vi "Runtest - Data Structure (FGV).vi"(7 "Action":T10=enum."Write", 8 "error in (no error)":errorcluster, 11 "Cluster In":T1={"Test Plan"=[], "PlanRow"=0, "Device Name"=[], "Timeout"=-1, "Start?"=FALSE, "Pause?"=FALSE, "IP Address"=[], "LogRow"=0, "Logtype"=0, "Log Elapse"=0.0, "Data"={"Station"="", "Sample ID"="", "Job No"="", "Job Description"="", "Filename"="", "Test Type"=0, "Speciment No"="", "Depth"="", "Height"="", "Diameter/Length"="", "Weight"="", "Test Parameter"="", "Station[]"=[], "Edit Pos"={"Row"=0, "Column"=0}, "Edit Pos Prev"={"Row"=0, "Column"=0}, "Area"="", "Path"="", "sample_id"=""}, "Stop log?"=FALSE, "tdms"=refnum, "Sensor Data"=[], "Start time"=timestamp(0 s since 1904-01-01), "Prev Log Elapse"=0, "Plot"=0, "X-Axis"=[0, 0, 0, 0], "Y-Axis"=[0, 0, 0, 0], "XY"=[], "End Stage?"=FALSE, "1run"=FALSE, "Condition"=[], "Start Con"=TRUE, "Log Con"=FALSE, "Stop Con"=FALSE, "Start Elapse"=0.0, "Start Load"=0.0, "Motor"=0, "StartRow"=0, "number log"=0, "Dir"=FALSE, "Start time test"=timestamp(0 s since 1904-01-01), "Auto"=FALSE, "Check return?"=FALSE, "Inv"={"M"=[], "Bool"=[]}, "tdms temp"=refnum, "Zero?"=FALSE, "Plot Timer"=0.0, "1st Run"=FALSE, "TDMS Path"=path "", "MaxLoad"=0.0, "Log Timer"=[], "Test Type"=0, "Log Sensor"=[], "Save?"=FALSE, "1st Log"=FALSE, "Y-Axis 2"=[], "On Y-Axis 2"=FALSE, "Decimal"=[], "Init"={"PWP TS"=0.0, "Load TS"=0.0, "Volume TS"=0.0, "Disp TS"=0.0, "CP"=0.0, "Vol In"=0.0, "Vol Out"=0.0, "Load UCT"=0.0, "Disp UCT"=0.0, "PWP Sat"=0.0, "CP Sat"=0.0, "Volume IsoCons"=0.0, "PWP IsoCons"=0.0, "PWP TUU"=0.0, "Load TUU"=0.0, "Volume TUU"=0.0, "Disp TUU"=0.0, "Load Cons"=0.0, "Disp Cons"=0.0, "Volume Sat"=0.0, "Vertical Load SB"=0.0, "Vertical Disp SB"=0.0, "H Disp SB"=0.0, "H Load SB"=0.0, "PWP BC"=0.0, "CP BC"=0.0, "PWP Sat Step"=0.0, "CP Sat Step"=0.0, "Volume Sat Step"=0.0, "PWP Sat Ramp"=0.0, "CP Sat Ramp"=0.0, "Volume Sat Ramp"=0.0}, "Calc"={"TS"={"Change PWP"=0.0, "Change Vol"=0.0, "Axial Load"=0.0, "CiL"=0.0, "Deviator"=0.0, "Axial Strain"=0.0, "MaxDeviator"=0.0, "SS"=0.0, "CAS"=0.0}, "TUU"={"Change PWP"=0.0, "Axial Load"=0.0, "CiL"=0.0, "Deviator"=0.0, "Axial Strain"=0.0, "MaxDeviator"=0.0}, "Sat"={"B Value"=0.0, "PWP Diss"=0.0, "CPP"=0.0, "CV"=0.0}, "Per"={"Change Vol In"=0.0, "Change Vol Out"=0.0, "Mean Vol"=0.0, "Gradient Pressure"=0.0, "Outlet Flow"=0.0, "Inlet Flow"=0.0, "I X1"=0.0, "I X2"=0.0, "I Y1"=0.0, "I Y2"=0.0, "O X1"=0.0, "O X2"=0.0, "O Y1"=0.0, "O Y2"=0.0}, "Step Cons"={"V Stress"=0.0, "H Settlement"=0.0, "Total H Settle"=0.0, "Prev Total H"=0.0}, "UCT"={"ALC"=0.0, "H Change"=0.0, "Deviator"=0.0, "Axial Strain"=0.0, "V Stress"=0.0, "MaxDeviator"=0.0}, "ISO Cons"={"CPP"=0.0, "PWP Diss"=0.0, "CV"=0.0, "VS"=0.0}, "SB"={"Speci LenC"=0.0, "Shear Strain"=0.0, "H LC"=0.0, "Normal Stress"=0.0, "Shear Stress"=0.0, "MaxShear"=0.0}, "BC"={"B Value"=0.0, "PWP Diss"=0.0, "CPP"=0.0, "CV"=0.0}, "Sat Step"={"B Value"=0.0, "PWP Diss"=0.0, "CPP"=0.0, "CV"=0.0}, "Sat Ramp"={"B Value"=0.0, "PWP Diss"=0.0, "CPP"=0.0, "CV"=0.0}}, "Device Index"=[], "Channel Index"=[], "http ref"=refnum, "fileid"="", "Step Cons"={"V Stress"=0.0, "H Settlement"=0.0}, "RunTest"=FALSE, "Graph Last"=0, "Init?"=FALSE, "Datalog"=[], "Start"={"Cons"={"VS"=0.0, "Delay"=FALSE, "No Delay"=0.0}, "Sat"={"CP"=0.0, "BP"=0.0, "StartBP"=FALSE, "Target CP"=FALSE, "Target BP"=FALSE}, "Iso"={"Select"=0.0, "BP"=0.0, "IC2"=0.0, "IC3"=0.0, "IC4"=0.0, ". IC6"=FALSE, "IC6"=0.0, "IC6-2"=0.0, "Time Cond"=0.0, "Last PWP"=0.0, "Target CP"=FALSE, "Target BP"=FALSE, "NewCP"=0.0, "NewBP"=0.0, "Noti CP"=FALSE, "Noti BP"=FALSE, "Noti PWP"=FALSE, "PrevSatBP"=0.0}, "TS"={"SS"=0.0, "Engage"=FALSE, "ES"=0.0, "LC"=0.0, "PreStart"=FALSE, "Trig SS"=FALSE, "Drain"=0.0, "Select"=0, "Max SS ."=FALSE, "MaxSS"=0.0}, "TUU"={"SS"=0.0, "Engage"=FALSE, "ES"=0.0, "LC"=0.0, "PreStart"=FALSE, "Trig SS"=FALSE, "CP"=0.0, "Delay Value"=0.0, "Delay"=FALSE, "CP PID"=FALSE}, "UCT"={"SS"=0.0, "Engage"=FALSE, "ES"=0.0, "LC"=0.0, "PreStart"=FALSE, "Trig SS"=FALSE}, "Enable?"=FALSE, "SB"={"SS"=0.0, "Engage"=FALSE, "ES"=0.0, "LC"=0.0, "PreStart"=FALSE, "Trig SS"=FALSE, "VS"=0.0, "Delay Value"=0.0, "Delay"=FALSE, "VS PID"=FALSE}, "Perm"={"DP"=0.0}, "BC"={"CP"=0.0, "Target CP"=FALSE, "Target BP"=FALSE, "CP Inc"=0.0, "CP .Init"=FALSE, "CP Init"=0.0, "1st BC"=FALSE}, "Sat (Step)"={"Select"=0.0, "CP"=0.0, "BP"=0.0, "EP"=0.0, "StartCP"=FALSE, "Target CP"=FALSE, "Target BP"=FALSE}, "Sat (Ramp)"={"Select"=0.0, "CP"=0.0, "BP"=0.0, "EP"=0.0, "StartCP"=FALSE, "Target CP"=FALSE, "Target BP"=FALSE, "Time Rate"=0}}, "Stop"={"Cons"={"Select"=0, "Disp"=0.0, "Time"=0.0, "Time2"=0.0, "Disp 2"=0.0, "Time Cond"=0.0, "Last Disp"=0.0, "Swell"=FALSE, "T50,90,100"={"t50_x_min"=0.0, "t50_y_value"=0.0, "t90_x_min"=0.0, "t90_y_value"=0.0, "t100_x_min"=0.0, "t100_y_value"=0.0, "target_column"="", "test_type"="", "error"=""}}, "Sat"={"Select"=0, "PP"=0.0, "Time"=0.0, "VC"=0.0, "Time2"=0.0, "Time Cond"=0.0, "Last PP"=0.0, ".B"=FALSE, "B"=0.0, "Last Vc"=0.0, "Time Cond 2"=0.0, "Time3"=0.0, "Time Cond 3"=0.0, "B Achieve"=FALSE, "PP Achieve"=FALSE, "VC Achieve"=FALSE, "Max Achieve"=FALSE, "CP Check"=0.0, "Skip Next"=FALSE, "B Achieve Stage"=0, ".CP Check"=FALSE}, "Iso"={"PP"=0.0, "Time"=0.0, "VC"=0.0, "Time2"=0.0, "Time Cond"=0.0, "Last Vc"=0.0, ".PP"=FALSE, "Time Cond 2"=0.0, "Select"=0, "BS"={"t50_x_min"=0.0, "t50_y_value"=0.0, "t90_x_min"=0.0, "t90_y_value"=0.0, "t100_x_min"=0.0, "t100_y_value"=0.0, "target_column"="", "test_type"="", "error"=""}, "Final VC"=0.0, "ASTM"={"t50_x_min"=0.0, "t50_y_value"=0.0, "t90_x_min"=0.0, "t90_y_value"=0.0, "t100_x_min"=0.0, "t100_y_value"=0.0, "target_column"="", "test_type"="", "error"=""}, "ASTM Log"={"t50_x_min"=0.0, "t50_y_value"=0.0, "t90_x_min"=0.0, "t90_y_value"=0.0, "t100_x_min"=0.0, "t100_y_value"=0.0, "target_column"="", "test_type"="", "error"=""}, "PP Achieve"=FALSE, "VC Achieve"=FALSE}, "TS"={"Axial"=0.0, ".MaxDev"=FALSE, "MaxDev Value"=0.0, "Return"=FALSE, "Reset"=FALSE, "Prev Time"=0.0, "PostStop Run"=FALSE, "CP Stop"=FALSE, "BP Stop"=FALSE, "PostStop Trig"=FALSE, "Reset Value"=0.0, "BPTrig"=FALSE, "CPTrig"=FALSE, "VLCTrig"=FALSE, "CAxial"=0.0, "Select"=0}, "TUU"={"Axial"=0.0, ".MaxDev"=FALSE, "MaxDev Value"=0.0, "Return"=FALSE, "Reset"=FALSE, "Prev Time"=0.0, "PostStop Run"=FALSE, "CP Stop"=FALSE, "BP Stop"=FALSE, "PostStop Trig"=FALSE, "Reset Value"=0.0, "BPTrig"=FALSE, "CPTrig"=FALSE, "VLCTrig"=FALSE}, "UCT"={"Axial"=0.0, ".MaxDev"=FALSE, "MaxDev Value"=0.0, "Return"=FALSE, "Reset"=FALSE, "Prev Time"=0.0, "PostStop Run"=FALSE, "CP Stop"=FALSE, "BP Stop"=FALSE, "PostStop Trig"=FALSE}, "Enable?"=FALSE, "SB"={"Shear"=0.0, ".MaxShear"=FALSE, "MaxShear Value"=0.0, "Return"=FALSE, "Reset"=FALSE, "Prev Time"=0.0, "PostStop Run"=FALSE, "CP Stop"=FALSE, "BP Stop"=FALSE, "PostStop Trig"=FALSE, "Reset Value"=0.0, "BPTrig"=FALSE, "CPTrig"=FALSE, "VLCTrig"=FALSE}, "Perm"={"Max Time"=FALSE, "Reset"=FALSE, "PostStop Run"=FALSE, "Ratio"=FALSE, "Reset Value"=0.0, "Time"=0.0, "RatioTime"=0.0, "RatioMore"=0.0, "RatioLess"=0.0, "Time Cond"=0.0, "Time Cond 2"=0.0, "Prev IF"=0.0, "Prev OF"=0.0, "PostStop Trig"=FALSE, "BP Trig"=FALSE, "DP Stop"=FALSE, "BP Stop"=FALSE, "CP Stop"=FALSE, "CP Trig"=FALSE}, "SP"={".Max Time"=FALSE, ".Time"=FALSE, "Time"=0.0, "MaxTime"=0.0, "Time Cond"=0.0, "Max Time Cond"=0.0, "Stress"=0.0}, "BC"={"Select"=0, "PP"=0.0, "Time"=0.0, "Time Cond"=0.0, "Last PP"=0.0, ".B"=FALSE, "B"=0.0, "Time 2"=0.0, "Time Cond 2"=0.0, "B Achieve"=FALSE, "PP Achieve"=FALSE, "Max Achieve"=FALSE, "CP Check"=0.0, "Skip Next"=FALSE, "B Achieve Stage"=0, ".CP Check"=FALSE}, "Sat (Step)"={"Select"=0, "PP"=0.0, "Time"=0.0, "VC"=0.0, "Time2"=0.0, "Time Cond"=0.0, "Last PP"=0.0, ".B"=FALSE, "B"=0.0, "Last Vc"=0.0, "Time Cond 2"=0.0, "Time3"=0.0, "Time Cond 3"=0.0, "B Achieve"=FALSE, "PP Achieve"=FALSE, "VC Achieve"=FALSE, "Max Achieve"=FALSE, "CP Check"=0.0, "Skip Next"=FALSE, "B Achieve Stage"=0}, "Sat (Ramp)"={"Select"=0, "PP"=0.0, "Time"=0.0, "VC"=0.0, "Time2"=0.0, "Time Cond"=0.0, "Last PP"=0.0, ".B"=FALSE, "B"=0.0, "Last Vc"=0.0, "Time Cond 2"=0.0, "Time3"=0.0, "Time Cond 3"=0.0, "B Achieve"=FALSE, "PP Achieve"=FALSE, "VC Achieve"=FALSE, "Max Achieve"=FALSE, "CP Check"=0.0, "Skip Next"=FALSE, "B Achieve Stage"=0}}, "Running?"=FALSE, "StartTime"=0.0, "Log Prev Time"=0.0, "KeyName"=[], "Test RunTime"=0.0, "Log Prev Axial"=0.0, "M Event"=[], "Last Log"=FALSE, "popup"=FALSE, "PreStart UU"=FALSE, "PreStart Sat"=FALSE, "PreStart BC"=FALSE, "PreStart Sat Step"=FALSE, "PreStart Sat Ramp"=FALSE, "Prev Sat IP"=""} {"M Event" items=["Stop", "Running", "PID", "Up Limit", "Down Limit", "Load Limit"]; "Test Type" items=["Please Select", "Triaxial Shear", "Triaxial UU", "Shearbox", "Permeability", "Consolidation (Stepped Loading)/Swelling", "Saturation (Incremental)", "User Defined", "UCT", "Isotropic Consolidation", "Swelling Pressure", "B-Check", "Saturation (Step Increment)", "Saturation (Ramp)"]; "Data"."Test Type" items=["Please Select", "Triaxial Shear", "Triaxial UU", "Shearbox", "Permeability", "Consolidation (Stepped Loading)/Swelling", "Saturation (Incremental)", "User Defined", "UCT", "Isotropic Consolidation", "Swelling Pressure", "B-Check", "Saturation (Step Increment)", "Saturation (Ramp)"]}) -> (0 "error out":errorcluster, 3 "Cluster Out":T1 {"M Event" items=["Stop", "Running", "PID", "Up Limit", "Down Limit", "Load Limit"]; "Test Type" items=["Please Select", "Triaxial Shear", "Triaxial UU", "Shearbox", "Permeability", "Consolidation (Stepped Loading)/Swelling", "Saturation (Incremental)", "User Defined", "UCT", "Isotropic Consolidation", "Swelling Pressure", "B-Check", "Saturation (Step Increment)", "Saturation (Ramp)"]; "Data"."Test Type" items=["Please Select", "Triaxial Shear", "Triaxial UU", "Shearbox", "Permeability", "Consolidation (Stepped Loading)/Swelling", "Saturation (Incremental)", "User Defined", "UCT", "Isotropic Consolidation", "Swelling Pressure", "B-Check", "Saturation (Step Increment)", "Saturation (Ramp)"]})   [LabVIEW 2019]
uses:
  Controls/FGV States.ctl
  Controls/RunTest - Data Structure.ctl
  Controls/Test Panel - Data Structure.ctl
  Controls/Station - Test Type.ctl
  <vilib>/Utility/miscctls.llb/LVRowAndColumnTypeDef.ctl
  Controls/RunTest - Calculate Data.ctl
  <vilib>/httpClient/ClientHandle.ctl
  Controls/RunTest - Start Condition.ctl
  Controls/RunTest - Stop Condition.ctl
  Controls/UDP - Event.ctl
  <vilib>/httpClient/LabVIEWHTTPClient.lvlib
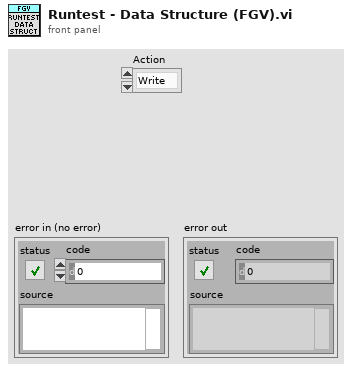
[diagram p1: front panel]
types:
  T1 = typedef "RunTest - Data Structure.ctl" = cluster{"Test Plan":string[], "PlanRow":i32, "Device Name":string[], "Timeout":i32, "Start?":bool, "Pause?":bool, "IP Address":string[], "LogRow":i32, "Logtype":u16, "Log Elapse":sgl, "Data":T2, "Stop log?":bool, "tdms":refnum<k34>, "Sensor Data":sgl[], "Start time":timestamp, "Prev Log Elapse":u32, "Plot":u16, "X-Axis":u16[], "Y-Axis":u16[], "XY":cluster{"X":dbl, "Y":dbl}[][], "End Stage?":bool, "1run":bool, "Condition":u16[], "Start Con":bool, "Log Con":bool, "Stop Con":bool, "Start Elapse":dbl, "Start Load":dbl, "Motor":i32, "StartRow":i32, "number log":i32, "Dir":bool, "Start time test":timestamp, "Auto":bool, "Check return?":bool, "Inv":cluster{"M":i32[], "Bool":bool[]}, "tdms temp":refnum<k34>, "Zero?":bool, "Plot Timer":dbl, "1st Run":bool, "TDMS Path":path, "MaxLoad":dbl, "Log Timer":sgl[], "Test Type":T3, "Log Sensor":string[], "Save?":bool, "1st Log":bool, "Y-Axis 2":u16[], "On Y-Axis 2":bool, "Decimal":u8[], "Init":cluster{"PWP TS":sgl, "Load TS":sgl, "Volume TS":sgl, "Disp TS":sgl, "CP":sgl, "Vol In":sgl, "Vol Out":sgl, "Load UCT":sgl, "Disp UCT":sgl, "PWP Sat":sgl, "CP Sat":sgl, "Volume IsoCons":sgl, "PWP IsoCons":sgl, "PWP TUU":sgl, "Load TUU":sgl, "Volume TUU":sgl, "Disp TUU":sgl, "Load Cons":sgl, "Disp Cons":sgl, "Volume Sat":sgl, "Vertical Load SB":sgl, "Vertical Disp SB":sgl, "H Disp SB":sgl, "H Load SB":sgl, "PWP BC":sgl, "CP BC":sgl, "PWP Sat Step":sgl, "CP Sat Step":sgl, "Volume Sat Step":sgl, "PWP Sat Ramp":sgl, "CP Sat Ramp":sgl, "Volume Sat Ramp":sgl}, "Calc":T5, "Device Index":i32[], "Channel Index":i32[], "http ref":T6, "fileid":string, "Step Cons":cluster{"V Stress":sgl, "H Settlement":sgl}, "RunTest":bool, "Graph Last":i32, "Init?":bool, "Datalog":bool[], "Start":T7, "Stop":T8, "Running?":bool, "StartTime":dbl, "Log Prev Time":dbl, "KeyName":string[], "Test RunTime":dbl, "Log Prev Axial":dbl, "M Event":T9[], "Last Log":bool, "popup":bool, "PreStart UU":bool, "PreStart Sat":bool, "PreStart BC":bool, "PreStart Sat Step":bool, "PreStart Sat Ramp":bool, "Prev Sat IP":string}
  T2 = typedef "Test Panel - Data Structure.ctl" = cluster{"Station":string, "Sample ID":string, "Job No":string, "Job Description":string, "Filename":string, "Test Type":T3, "Speciment No":string, "Depth":string, "Height":string, "Diameter/Length":string, "Weight":string, "Test Parameter":string, "Station[]":string[], "Edit Pos":T4, "Edit Pos Prev":T4, "Area":string, "Path":string, "sample_id":string}
  T3 = typedef "Station - Test Type.ctl" = u16
  T4 = typedef "LVRowAndColumnTypeDef.ctl" = cluster{"Row":i32, "Column":i32}
  T5 = typedef "RunTest - Calculate Data.ctl" = cluster{"TS":cluster{"Change PWP":sgl, "Change Vol":sgl, "Axial Load":sgl, "CiL":sgl, "Deviator":sgl, "Axial Strain":sgl, "MaxDeviator":sgl, "SS":sgl, "CAS":sgl}, "TUU":cluster{"Change PWP":sgl, "Axial Load":sgl, "CiL":sgl, "Deviator":sgl, "Axial Strain":sgl, "MaxDeviator":sgl}, "Sat":cluster{"B Value":sgl, "PWP Diss":sgl, "CPP":sgl, "CV":sgl}, "Per":cluster{"Change Vol In":sgl, "Change Vol Out":sgl, "Mean Vol":sgl, "Gradient Pressure":sgl, "Outlet Flow":sgl, "Inlet Flow":sgl, "I X1":sgl, "I X2":sgl, "I Y1":sgl, "I Y2":sgl, "O X1":sgl, "O X2":sgl, "O Y1":sgl, "O Y2":sgl}, "Step Cons":cluster{"V Stress":sgl, "H Settlement":sgl, "Total H Settle":sgl, "Prev Total H":sgl}, "UCT":cluster{"ALC":sgl, "H Change":sgl, "Deviator":sgl, "Axial Strain":sgl, "V Stress":sgl, "MaxDeviator":sgl}, "ISO Cons":cluster{"CPP":sgl, "PWP Diss":sgl, "CV":sgl, "VS":sgl}, "SB":cluster{"Speci LenC":sgl, "Shear Strain":sgl, "H LC":sgl, "Normal Stress":sgl, "Shear Stress":sgl, "MaxShear":sgl}, "BC":cluster{"B Value":sgl, "PWP Diss":sgl, "CPP":sgl, "CV":sgl}, "Sat Step":cluster{"B Value":sgl, "PWP Diss":sgl, "CPP":sgl, "CV":sgl}, "Sat Ramp":cluster{"B Value":sgl, "PWP Diss":sgl, "CPP":sgl, "CV":sgl}}
  T6 = typedef "LabVIEWHTTPClient.lvlib/ClientHandle.ctl" = refnum<k1>
  T7 = typedef "RunTest - Start Condition.ctl" = cluster{"Cons":cluster{"VS":dbl, "Delay":bool, "No Delay":dbl}, "Sat":cluster{"CP":dbl, "BP":dbl, "StartBP":bool, "Target CP":bool, "Target BP":bool}, "Iso":cluster{"Select":dbl, "BP":dbl, "IC2":dbl, "IC3":dbl, "IC4":dbl, ". IC6":bool, "IC6":dbl, "IC6-2":dbl, "Time Cond":dbl, "Last PWP":dbl, "Target CP":bool, "Target BP":bool, "NewCP":dbl, "NewBP":dbl, "Noti CP":bool, "Noti BP":bool, "Noti PWP":bool, "PrevSatBP":dbl}, "TS":cluster{"SS":dbl, "Engage":bool, "ES":dbl, "LC":dbl, "PreStart":bool, "Trig SS":bool, "Drain":dbl, "Select":u16, "Max SS .":bool, "MaxSS":dbl}, "TUU":cluster{"SS":dbl, "Engage":bool, "ES":dbl, "LC":dbl, "PreStart":bool, "Trig SS":bool, "CP":dbl, "Delay Value":dbl, "Delay":bool, "CP PID":bool}, "UCT":cluster{"SS":dbl, "Engage":bool, "ES":dbl, "LC":dbl, "PreStart":bool, "Trig SS":bool}, "Enable?":bool, "SB":cluster{"SS":dbl, "Engage":bool, "ES":dbl, "LC":dbl, "PreStart":bool, "Trig SS":bool, "VS":dbl, "Delay Value":dbl, "Delay":bool, "VS PID":bool}, "Perm":cluster{"DP":dbl}, "BC":cluster{"CP":dbl, "Target CP":bool, "Target BP":bool, "CP Inc":dbl, "CP .Init":bool, "CP Init":dbl, "1st BC":bool}, "Sat (Step)":cluster{"Select":dbl, "CP":dbl, "BP":dbl, "EP":dbl, "StartCP":bool, "Target CP":bool, "Target BP":bool}, "Sat (Ramp)":cluster{"Select":dbl, "CP":dbl, "BP":dbl, "EP":dbl, "StartCP":bool, "Target CP":bool, "Target BP":bool, "Time Rate":u32}}
  T8 = typedef "RunTest - Stop Condition.ctl" = cluster{"Cons":cluster{"Select":i32, "Disp":dbl, "Time":dbl, "Time2":dbl, "Disp 2":dbl, "Time Cond":dbl, "Last Disp":dbl, "Swell":bool, "T50,90,100":cluster{"t50_x_min":dbl, "t50_y_value":dbl, "t90_x_min":dbl, "t90_y_value":dbl, "t100_x_min":dbl, "t100_y_value":dbl, "target_column":string, "test_type":string, "error":string}}, "Sat":cluster{"Select":i32, "PP":dbl, "Time":dbl, "VC":dbl, "Time2":dbl, "Time Cond":dbl, "Last PP":dbl, ".B":bool, "B":dbl, "Last Vc":dbl, "Time Cond 2":dbl, "Time3":dbl, "Time Cond 3":dbl, "B Achieve":bool, "PP Achieve":bool, "VC Achieve":bool, "Max Achieve":bool, "CP Check":dbl, "Skip Next":bool, "B Achieve Stage":u32, ".CP Check":bool}, "Iso":cluster{"PP":dbl, "Time":dbl, "VC":dbl, "Time2":dbl, "Time Cond":dbl, "Last Vc":dbl, ".PP":bool, "Time Cond 2":dbl, "Select":i32, "BS":cluster{"t50_x_min":dbl, "t50_y_value":dbl, "t90_x_min":dbl, "t90_y_value":dbl, "t100_x_min":dbl, "t100_y_value":dbl, "target_column":string, "test_type":string, "error":string}, "Final VC":dbl, "ASTM":cluster{"t50_x_min":dbl, "t50_y_value":dbl, "t90_x_min":dbl, "t90_y_value":dbl, "t100_x_min":dbl, "t100_y_value":dbl, "target_column":string, "test_type":string, "error":string}, "ASTM Log":cluster{"t50_x_min":dbl, "t50_y_value":dbl, "t90_x_min":dbl, "t90_y_value":dbl, "t100_x_min":dbl, "t100_y_value":dbl, "target_column":string, "test_type":string, "error":string}, "PP Achieve":bool, "VC Achieve":bool}, "TS":cluster{"Axial":dbl, ".MaxDev":bool, "MaxDev Value":dbl, "Return":bool, "Reset":bool, "Prev Time":dbl, "PostStop Run":bool, "CP Stop":bool, "BP Stop":bool, "PostStop Trig":bool, "Reset Value":dbl, "BPTrig":bool, "CPTrig":bool, "VLCTrig":bool, "CAxial":dbl, "Select":i32}, "TUU":cluster{"Axial":dbl, ".MaxDev":bool, "MaxDev Value":dbl, "Return":bool, "Reset":bool, "Prev Time":dbl, "PostStop Run":bool, "CP Stop":bool, "BP Stop":bool, "PostStop Trig":bool, "Reset Value":dbl, "BPTrig":bool, "CPTrig":bool, "VLCTrig":bool}, "UCT":cluster{"Axial":dbl, ".MaxDev":bool, "MaxDev Value":dbl, "Return":bool, "Reset":bool, "Prev Time":dbl, "PostStop Run":bool, "CP Stop":bool, "BP Stop":bool, "PostStop Trig":bool}, "Enable?":bool, "SB":cluster{"Shear":dbl, ".MaxShear":bool, "MaxShear Value":dbl, "Return":bool, "Reset":bool, "Prev Time":dbl, "PostStop Run":bool, "CP Stop":bool, "BP Stop":bool, "PostStop Trig":bool, "Reset Value":dbl, "BPTrig":bool, "CPTrig":bool, "VLCTrig":bool}, "Perm":cluster{"Max Time":bool, "Reset":bool, "PostStop Run":bool, "Ratio":bool, "Reset Value":dbl, "Time":dbl, "RatioTime":dbl, "RatioMore":dbl, "RatioLess":dbl, "Time Cond":dbl, "Time Cond 2":dbl, "Prev IF":dbl, "Prev OF":dbl, "PostStop Trig":bool, "BP Trig":bool, "DP Stop":bool, "BP Stop":bool, "CP Stop":bool, "CP Trig":bool}, "SP":cluster{".Max Time":bool, ".Time":bool, "Time":dbl, "MaxTime":dbl, "Time Cond":dbl, "Max Time Cond":dbl, "Stress":dbl}, "BC":cluster{"Select":i32, "PP":dbl, "Time":dbl, "Time Cond":dbl, "Last PP":dbl, ".B":bool, "B":dbl, "Time 2":dbl, "Time Cond 2":dbl, "B Achieve":bool, "PP Achieve":bool, "Max Achieve":bool, "CP Check":dbl, "Skip Next":bool, "B Achieve Stage":u32, ".CP Check":bool}, "Sat (Step)":cluster{"Select":i32, "PP":dbl, "Time":dbl, "VC":dbl, "Time2":dbl, "Time Cond":dbl, "Last PP":dbl, ".B":bool, "B":dbl, "Last Vc":dbl, "Time Cond 2":dbl, "Time3":dbl, "Time Cond 3":dbl, "B Achieve":bool, "PP Achieve":bool, "VC Achieve":bool, "Max Achieve":bool, "CP Check":dbl, "Skip Next":bool, "B Achieve Stage":u32}, "Sat (Ramp)":cluster{"Select":i32, "PP":dbl, "Time":dbl, "VC":dbl, "Time2":dbl, "Time Cond":dbl, "Last PP":dbl, ".B":bool, "B":dbl, "Last Vc":dbl, "Time Cond 2":dbl, "Time3":dbl, "Time Cond 3":dbl, "B Achieve":bool, "PP Achieve":bool, "VC Achieve":bool, "Max Achieve":bool, "CP Check":dbl, "Skip Next":bool, "B Achieve Stage":u32}}
  T9 = typedef "UDP - Event.ctl" = u16
  T10 = typedef "FGV States.ctl" = enum16{"Read", "Write"}
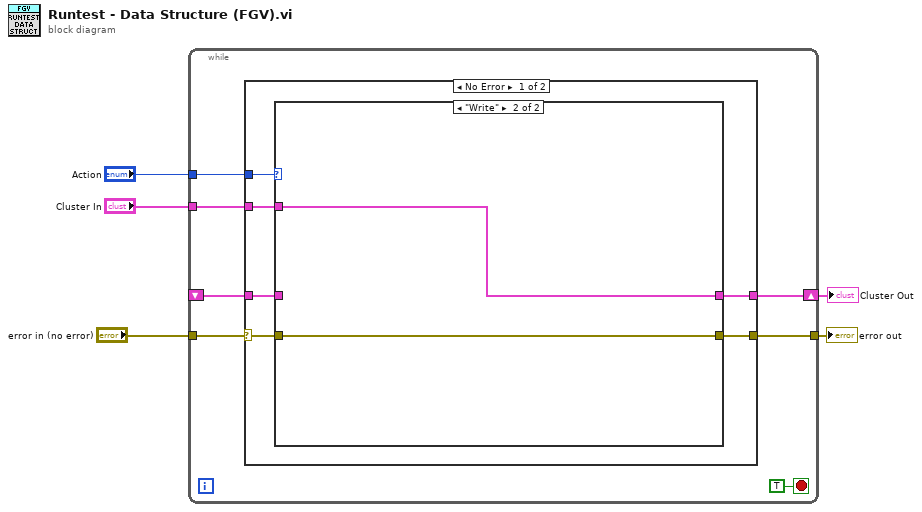
[diagram p0: block diagram]
diagram:
  n1 = while {
    tunnel: "Action" -> [w12]
    tunnel: "Cluster In" -> [w10]
    shift-right: [w11] -> w1
    shift-left: _ -> [w9]
    tunnel: "error in (no error)" -> [w7]
    tunnel: [w6] -> w3
    stop <- TRUE stop-if-true
    n2 = case shown="No Error" w7 {
      selector: w7 -> [w13 w23]
      tunnel: w12 -> [w18 _]
      tunnel: [w17 w24] -> w11
      tunnel: w10 -> [w16 _]
      tunnel: w9 -> [w15 w24]
      tunnel: [w14 w23] -> w6
      frame No Error {
        n3 = case shown="\"Write\"" w18 {
          tunnel: [w20 w22] -> w17
          tunnel: w16 -> [_ w22]
          tunnel: w15 -> [w20 _]
          tunnel: [w19 w21] -> w14
          tunnel: w13 -> [w19 w21]
          frame "Read", Default {
          }
          frame "Write" {
          }
        }
      }
      frame Error {
      }
    }
  }
  "error out" <- w3
  "Cluster Out" <- w1
